vi "B.vi"(0 "x":dbl, 11 "error in":errorcluster) -> (4 "y":dbl, 15 "error out":errorcluster)   [LabVIEW 2026]
doc: "Repro caller: calls A.vi."
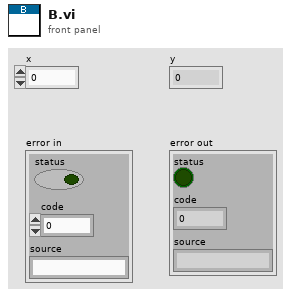
[diagram p1: front panel]
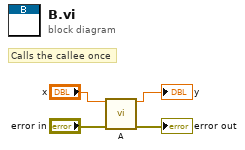
[diagram p0: block diagram]
diagram:
  # "Calls the callee once"
  n1 = call "A.vi"("x"="x", "error in"="error in") -> ("y"=→"y":dbl, "error out"=→"error out":errorcluster)  [unwired: 12 in]
